vi "updateScreen.vi"(0 "reference":refnum<class "Graphics.lvclass">, 5 "error in (no error)":errorcluster) -> (14 "reference out":refnum<class "Graphics.lvclass">, 17 "picture":picture, 19 "error out":errorcluster)   [LabVIEW 2020, in "Graphics.lvclass"]
doc: "Updates the screen"
uses:
  <resource>/Framework/Providers/Open_GDS/UML/Graphics_class/Graphics.lvclass
panel:
  out "x-y":u32
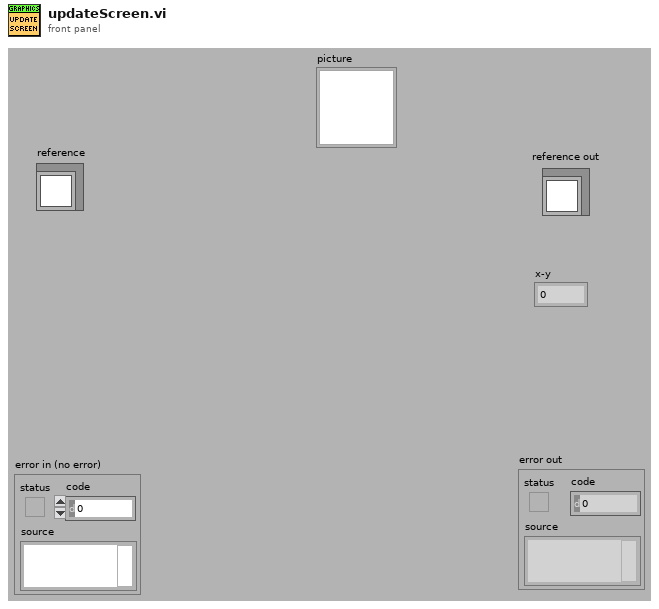
[diagram p1: front panel]
types:
  T1 = typedef "Graphics.lvclass/ObjectAttributes.ctl" = cluster{"drawColor":u32, "backgroundColor":u32, "font":T2, "fontType":T3, "picture":picture, "stroke":T4, "scaleX":dbl, "scaleY":dbl, "screenRef":refnum<vi>, "offsetX":dbl, "offsetY":dbl}
  T2 = typedef "Graphics.lvclass/FontType.ctl" = cluster{"Font Name:":string, "Size":i16, "Strikeout?":bool, "Italic?":bool, "Underline?":bool, "Outline?":bool, "Shadow?":bool, "Bold?":bool}
  T3 = typedef "Graphics.lvclass/LvFontType.ctl" = enum16{"User-specified Font", "Application Font", "System Font", "Dialog Font"}
  T4 = typedef "Graphics.lvclass/StrokeType.ctl" = enum16{"USE_DEFAULT", "SOLID", "DOTTED"}
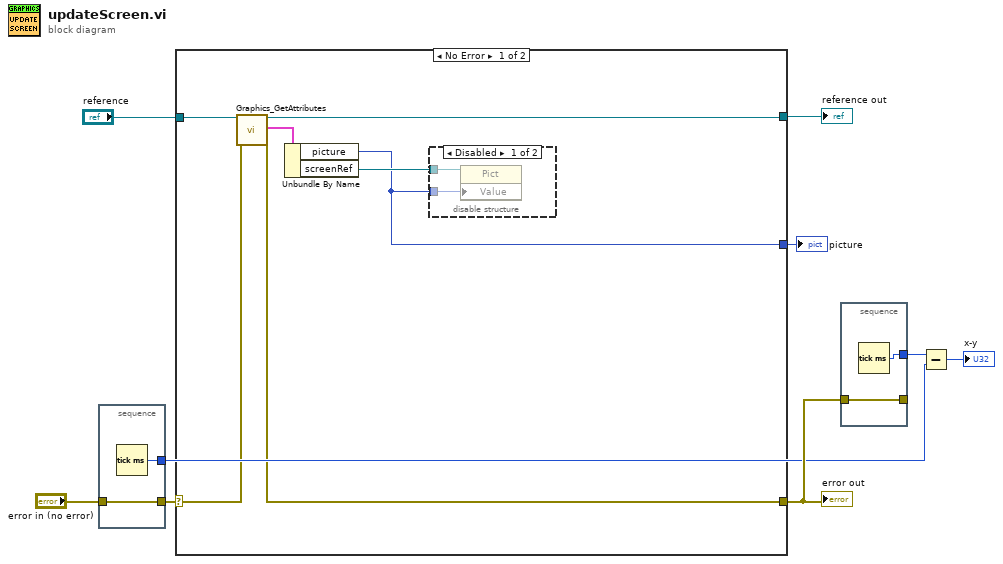
[diagram p0: block diagram]
diagram:
  n1 = stacked-sequence {
    tunnel: "error in (no error)" -> [w11]
    tunnel: [w11] -> w6
    tunnel: [w10] -> w3
    frame #0 {
      n2 = Tick Count (ms)() -> (millisecond timer value=w10:u32)
    }
  }
  n3 = case shown="No Error" w6 {
    selector: w6 -> [w18 w21]
    tunnel: "reference" -> [w17 w22]
    tunnel: [w15 w21] -> w5
    tunnel: [w16 w22] -> w8
    tunnel: [w12 _] -> w1
    frame No Error {
      n4 = call <resource>:"Graphics_GetAttributes.vi"("reference in"=w17, "error in (no error)"=w18) -> ("reference out"=w16:refnum<class "Graphics.lvclass">, "Data"=w13:T1, "error out"=w15:errorcluster)  [unwired: 1 in, 14 out]
      n5 = Unbundle By Name(w13) -> ("picture"=w12:picture, "screenRef"=w14:refnum<vi>)
      n6 = disable-structure shown="Disabled" {
        disable-tunnel: w14 -> [w20 _]
        disable-tunnel: w12 -> [w19 _]
        frame Disabled {
          n7 = property class="Pict"(reference=w20, "Value"=w19) -> ()  [unwired: 1 in, 2 out]
        }
        frame Enabled {
        }
      }
    }
    frame Error {
    }
  }
  "reference out" <- w8
  "error out" <- w5
  "picture" <- w1
  n8 = stacked-sequence {
    tunnel: w5 -> [w24]
    tunnel: [w24] -> _
    tunnel: [w23] -> w4
    frame #0 {
      n9 = Tick Count (ms)() -> (millisecond timer value=w23:u32)
    }
  }
  n10 = Subtract(x=w4, y=w3) -> (x-y=→"x-y":u32)
